vi "Signal Time Assigned Table.vi"(8 "time":dbl[](array[numeric]), 11 "Assinged Signal Profile plus":T1) -> (3 "Signal Profile Table":string[][](table) caption="表")   [LabVIEW 2018]
panel:
  in  "Signal Tag":string[](array[string])
  out "配列":string[][](array[string])
  out "要素":i32
  out "サイズ 3":i32
  out "サイズ 2":i32[](array[numeric])
  out "Signal Base Species C":i32[][](array[numeric])
  out "サイズ":i32
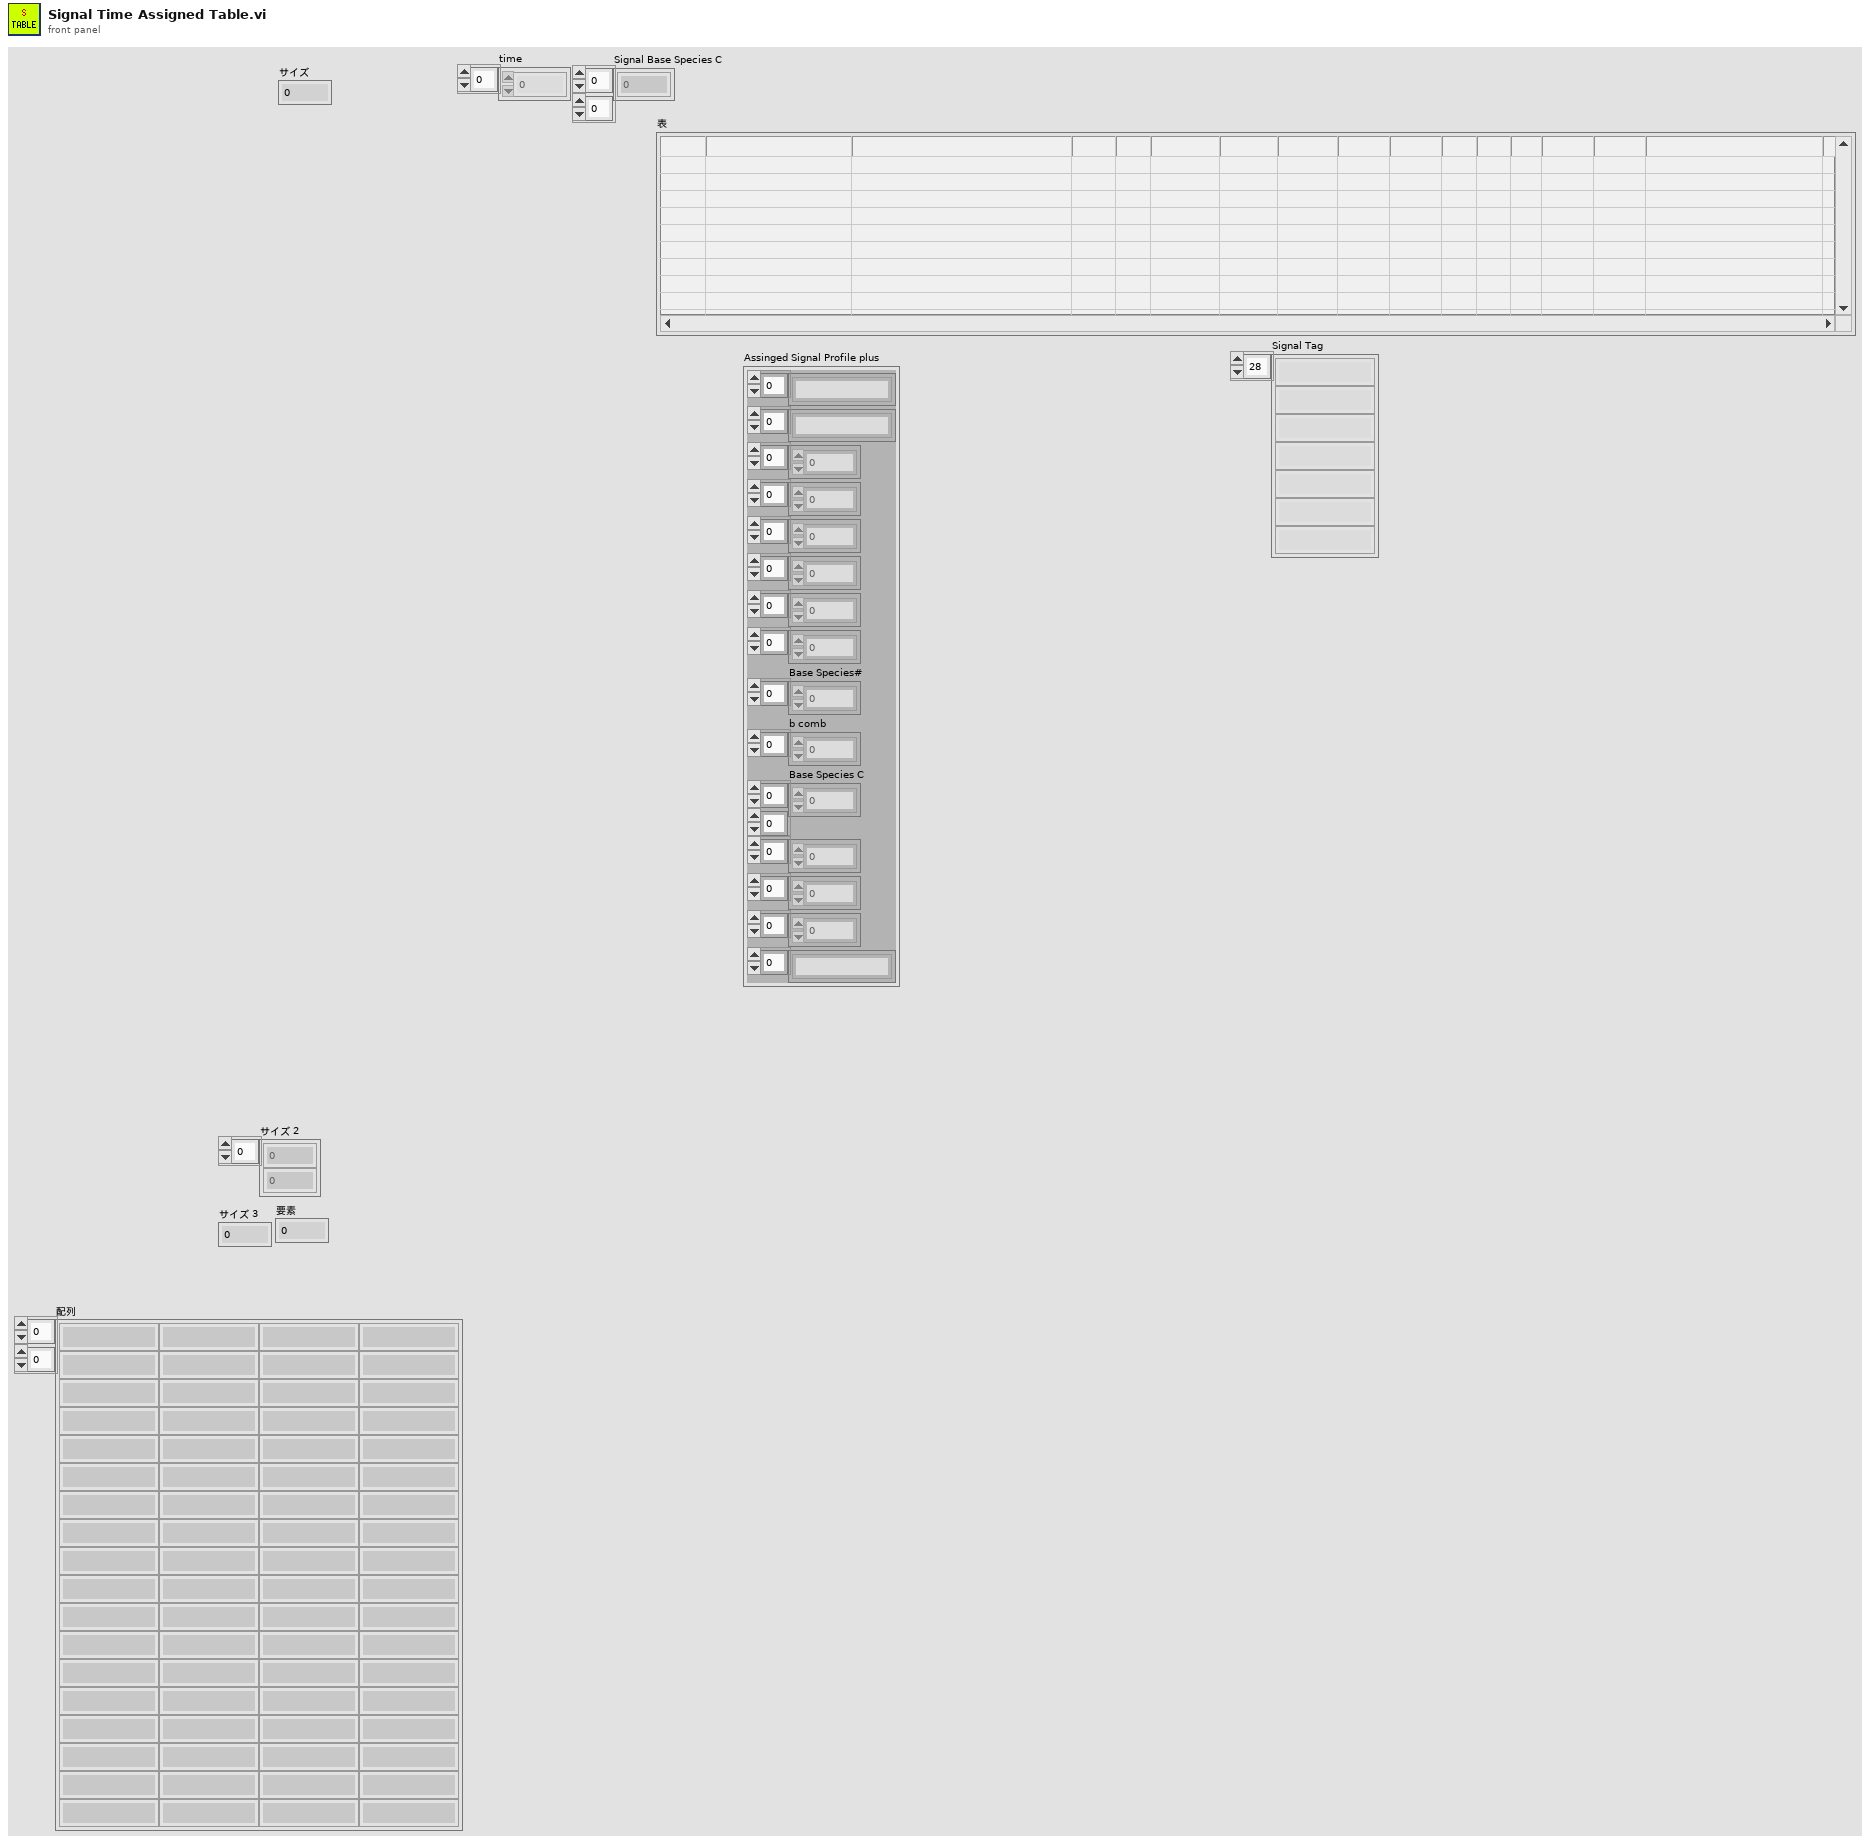
[diagram p1: front panel]
types:
  T1 = cluster{string[], string[], i32[], i32[], i32[], i32[], dbl[], dbl[], "Base Species#":i16[], "b comb":u32[], "Base Species C":i32[][], i32[], i32[], i32[], string[]}
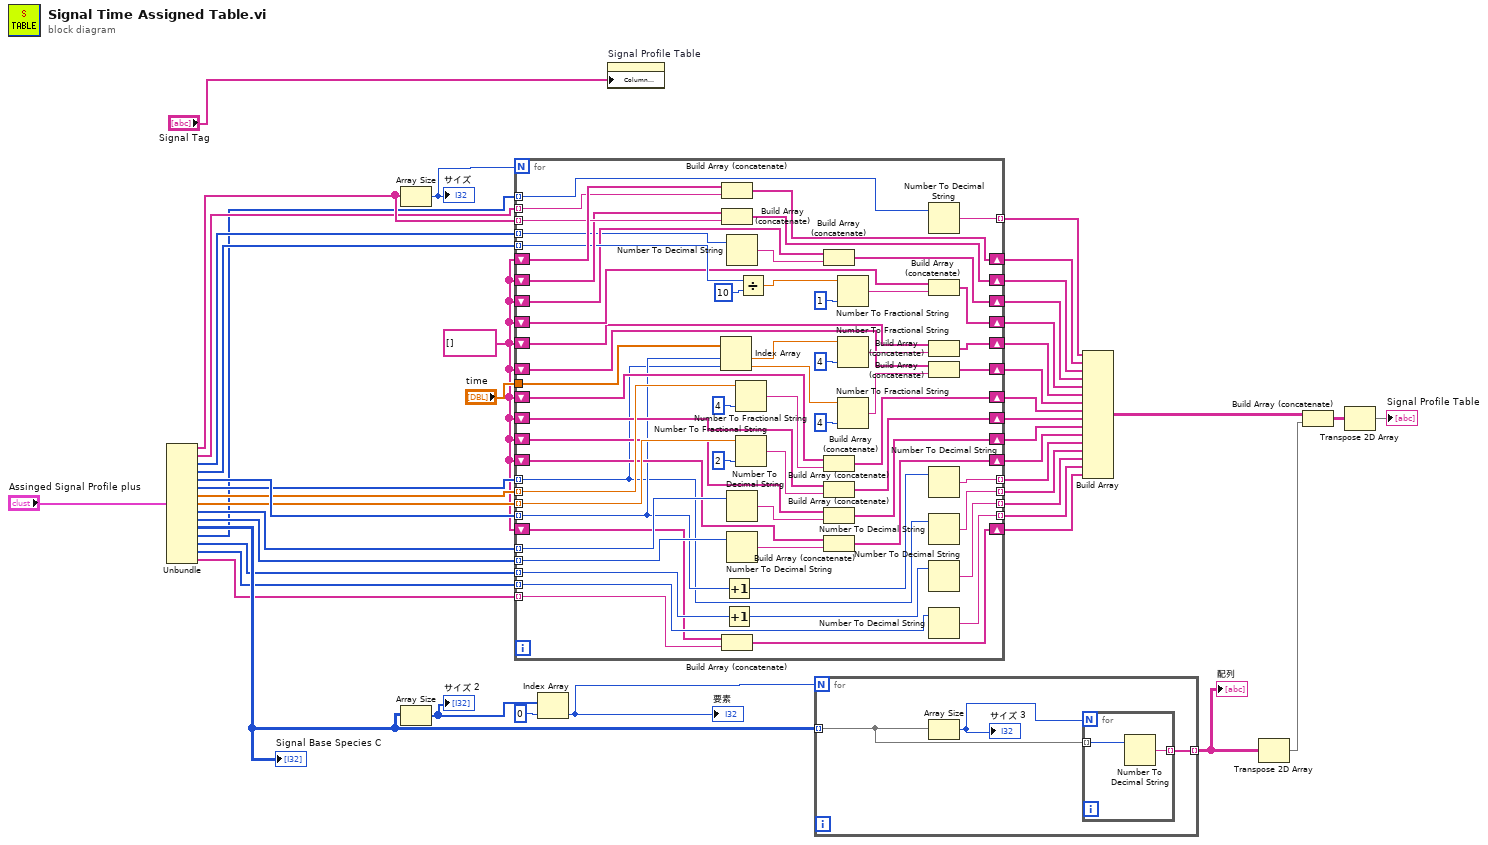
[diagram p0: block diagram]
diagram:
  w4 = string[] []
  n1 = Unbundle("Assinged Signal Profile plus") -> (w18:string[], w17:string[], w16:i32[], w15:i32[], w14:i32[], w13:i32[], w12:dbl[], w11:dbl[], "Base Species#"=w10:i16[], "b comb"=w9:u32[], "Base Species C"=w8:i32[][], w7:i32[], w6:i32[], w5:i32[], w3:string[])
  "Signal Base Species C" <- w8
  n2 = Array Size(array=w18) -> (size(s)=w44:i32)
  "サイズ" <- w44
  n3 = Array Size(array=w8) -> (size(s)=w31:i32[])
  "サイズ 2" <- w31
  n4 = for {
    N: w44 -> [_]
    tunnel: w18 -> [w93] mode=indexing
    tunnel: w17 -> [w94] mode=indexing
    tunnel: w16 -> [w69] mode=indexing
    tunnel: w15 -> [w87] mode=indexing
    tunnel: w14 -> [w57] mode=indexing
    tunnel: w13 -> [w55] mode=indexing
    tunnel: w12 -> [w98] mode=indexing
    tunnel: w11 -> [w97] mode=indexing
    tunnel: "time" -> [w105]
    shift-right: [w95] -> w42
    shift-left: w4 -> [w96]
    shift-right: [w92] -> w41
    shift-left: w4 -> [w91]
    shift-right: [w83] -> w40
    shift-left: w4 -> [w82]
    shift-right: [w81] -> w39
    shift-left: w4 -> [w80]
    shift-right: [w77] -> w38
    shift-left: w4 -> [w76]
    shift-right: [w75] -> w37
    shift-left: w4 -> [w74]
    shift-right: [w73] -> w36
    shift-left: w4 -> [w72]
    shift-right: [w71] -> w35
    shift-left: w4 -> [w70]
    tunnel: w10 -> [w67] mode=indexing
    tunnel: w9 -> [w66] mode=indexing
    shift-right: [w65] -> w33
    shift-left: w4 -> [w64]
    shift-right: [w62] -> w32
    shift-left: w4 -> [w61]
    tunnel: w7 -> [w59] mode=indexing
    tunnel: [w58] -> w24 mode=indexing
    tunnel: [w56] -> w23 mode=indexing
    tunnel: [w54] -> w22 mode=indexing
    tunnel: w6 -> [w53] mode=indexing
    tunnel: w5 -> [w52] mode=indexing
    tunnel: [w51] -> w21 mode=indexing
    tunnel: [w50] -> w20 mode=indexing
    shift-right: [w47] -> w2
    shift-left: w4 -> [w46]
    tunnel: w3 -> [w45] mode=indexing
    n5 = Index Array(array=w105, index #1=w57, index #2=w55) -> (element #1=w102:dbl, element #2=w101:dbl)
    n6 = Build Array (concatenate)(w96, w94) -> (w95:string[])
    n7 = Build Array (concatenate)(w91, w93) -> (w92:string[])
    n8 = Build Array (concatenate)(w46, w45) -> (w47:string[])
    n9 = Increment(x=w57) -> (x+1=w49:i32)
    n10 = Increment(x=w53) -> (x+1=w48:i32)
    n11 = Number To Decimal String(number=w69) -> (decimal integer string=w68:string)  [unwired: 1 in]
    n12 = Number To Decimal String(number=w67) -> (decimal integer string=w63:string)  [unwired: 1 in]
    n13 = Number To Decimal String(number=w66) -> (decimal integer string=w60:string)  [unwired: 1 in]
    n14 = Number To Fractional String(number=w98, precision (6)=i16 4 ("精度（6）")) -> (F-format string=w79:string)  [unwired: 2 in]
    n15 = Number To Fractional String(number=w97, precision (6)=i16 2 ("精度（6）")) -> (F-format string=w78:string)  [unwired: 2 in]
    n16 = Divide(x=w87, y=10) -> (x/y=w85:dbl)
    n17 = Build Array (concatenate)(w82, w68) -> (w83:string[])
    n18 = Build Array (concatenate)(w72, w79) -> (w73:string[])
    n19 = Build Array (concatenate)(w70, w78) -> (w71:string[])
    n20 = Build Array (concatenate)(w64, w63) -> (w65:string[])
    n21 = Build Array (concatenate)(w61, w60) -> (w62:string[])
    n22 = Number To Fractional String(number=w85, precision (6)=i16 1 ("精度（6）")) -> (F-format string=w84:string)  [unwired: 2 in]
    n23 = Number To Fractional String(number=w102, precision (6)=i16 4 ("精度（6）")) -> (F-format string=w90:string)  [unwired: 2 in]
    n24 = Number To Fractional String(number=w101, precision (6)=i16 4 ("精度（6）")) -> (F-format string=w89:string)  [unwired: 2 in]
    n25 = Number To Decimal String(number=w59) -> (decimal integer string=w58:string)  [unwired: 1 in]
    n26 = Build Array (concatenate)(w80, w84) -> (w81:string[])
    n27 = Build Array (concatenate)(w76, w90) -> (w77:string[])
    n28 = Build Array (concatenate)(w74, w89) -> (w75:string[])
    n29 = Number To Decimal String(number=w49) -> (decimal integer string=w56:string)  [unwired: 1 in]
    n30 = Number To Decimal String(number=w55) -> (decimal integer string=w54:string)  [unwired: 1 in]
    n31 = Number To Decimal String(number=w48) -> (decimal integer string=w51:string)  [unwired: 1 in]
    n32 = Number To Decimal String(number=w52) -> (decimal integer string=w50:string)  [unwired: 1 in]
  }
  n33 = Index Array(array=w31, index=0 ("指標")) -> (element=w29:i32)
  "要素" <- w29
  n34 = property on="Signal Profile Table" class="Tbl (strict)"("Column Headers[]"="Signal Tag") -> ()  [unwired: 2 in, 2 out]
  n35 = for {
    N: w29 -> [_]
    tunnel: w8 -> [w107] mode=indexing
    tunnel: [w106] -> w28 mode=indexing
    n36 = Array Size(array=w107) -> (size(s)=w108:i32)
    "サイズ 3" <- w108
    n37 = for {
      N: w108 -> [_]
      tunnel: w107 -> [w110] mode=indexing
      tunnel: [w109] -> w106 mode=indexing
      n38 = Number To Decimal String(number=w110) -> (decimal integer string=w109:string)  [unwired: 1 in]
    }
  }
  "配列" <- w28
  n39 = Build Array(w24, w42, w41, w40, w39, w38, w37, w36, w35, w33, w32, w23, w22, w21, w20, w2) -> (w27:string[][])
  n40 = Transpose 2D Array(2D array=w28) -> (transposed array=w25:string[][])
  n41 = Build Array (concatenate)(w27, w25) -> (w26:string[][])
  n42 = Transpose 2D Array(2D array=w26) -> (transposed array=→"Signal Profile Table":string[][])
